vi "linked-ignore-default.vi"(0 "Ignored default":path=path "C:/wirelint-fixture/ignored-default.txt", 5 "Reported default":path=path "C:/wirelint-fixture/reported-default.txt", 11 "error in":errorcluster) -> (15 "error out":errorcluster)   [LabVIEW 2024]
doc: "Data-only fixture for an ignore arrow from a block diagram path terminal to its front panel default. No file operations are performed."
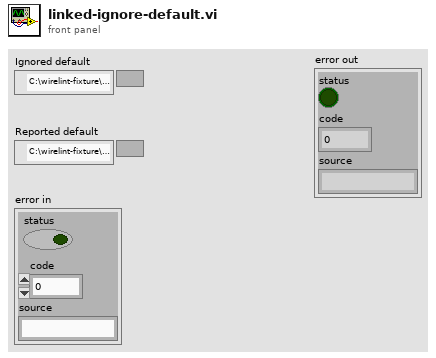
[diagram p1: front panel]
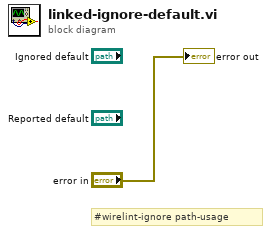
[diagram p0: block diagram]
diagram:
  # "#wirelint-ignore path-usage"
  "error out" <- "error in"
